vi "ADI_IMU_ADIS16448_Loop.vi"(8 "error in":errorcluster, 11 "ADI IMU DevRef":T1={"DevStatus"={"status"=FALSE, "code"=0, "source"=""}, "Handle"=0, "SPI Bus"=enum."SPI On-Board, CS0", "Device Found"=FALSE, "Device Ready"=FALSE, "Yaw Axis"=enum."Z", "AHRS Algorithm"=enum."Complementary", "Serial"=0, "Lot ID 2"=0, "Lot ID 1"=0, "Bytes Per Sample"=0, "Calibrate On Open?"=FALSE}) -> (1 "Device Found":bool)   [LabVIEW 2017, in "ADIS16448_IMU.lvlib"]
doc: "Periodically reads the ADI MXP IMU valuse and makes data available for use elsewhere in your robot project. Place this block within PeriodicTasks.vi outside any loops."
uses:
  ADIS16448_IMU.lvlib
  ADI_IMU_ADIS16448_IMUDevRef.ctl
  <vilib>/Rock Robotics/SystemInterfaces/spilib/spi_bus.ctl
panel:
  in  "Main Name":string
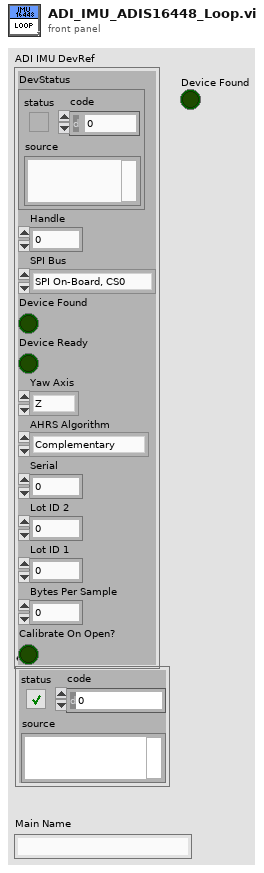
[diagram p1: front panel]
types:
  T1 = typedef "ADIS16448_IMU.lvlib/ADI_IMU_ADIS16448_IMUDevRef.ctl" = cluster{"DevStatus":errorcluster, "Handle":i32, "SPI Bus":T2, "Device Found":bool, "Device Ready":bool, "Yaw Axis":enum16{"X", "Y", "Z"}, "AHRS Algorithm":enum16{"Complementary", "Madgwick"}, "Serial":u16, "Lot ID 2":u16, "Lot ID 1":u16, "Bytes Per Sample":u16, "Calibrate On Open?":bool}
  T2 = typedef "spi_bus.ctl" = enum16{"SPI On-Board, CS0", "SPI On-Board, CS1", "SPI On-Board, CS2", "SPI On-Board, CS3", "SPI MXP", "Invalid"}
  T3 = cluster{"X Angle":dbl, "Y Angle":dbl, "Z Angle":dbl}
  T4 = enum32{"Bad", "Idle", "Run top level", "Running"}
  T5 = cluster{"X Gyro":dbl, "Y Gyro":dbl, "Z Gyro":dbl, "X Accel":dbl, "Y Accel":dbl, "Z Accel":dbl, "X Mag":dbl, "Y Mag":dbl, "Z Mag":dbl, "Pressure":dbl, "Temp":dbl}
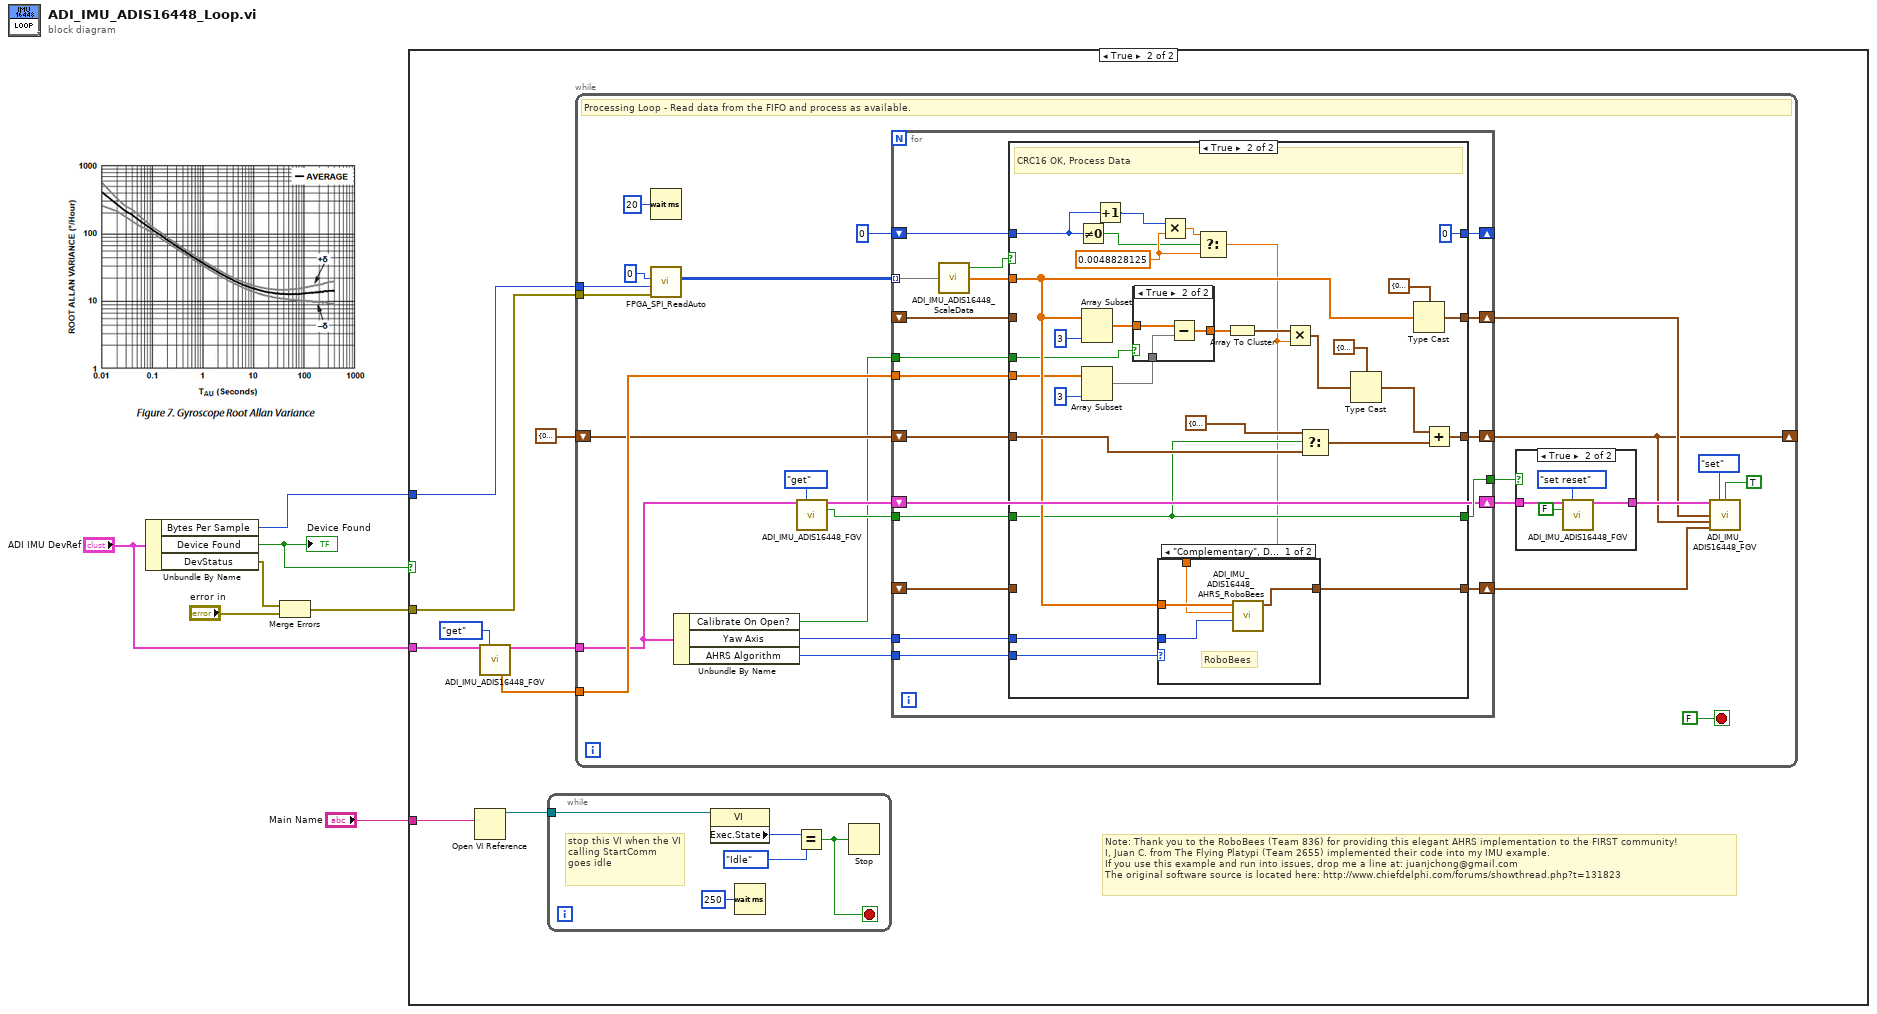
[diagram p0: block diagram]
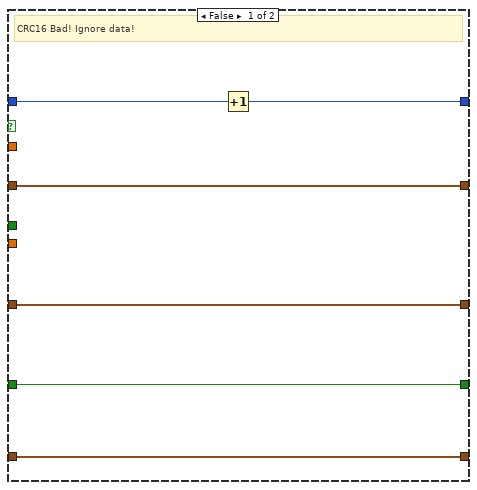
[diagram p3: hidden frame]
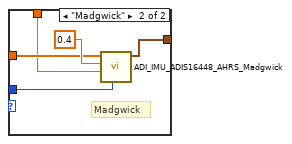
[diagram p5: hidden frame]
diagram:
  n1 = Unbundle By Name("ADI IMU DevRef") -> ("Bytes Per Sample"=w2:u16, "Device Found"=w4:bool, "DevStatus"=w5:errorcluster)
  "Device Found" <- w4
  n2 = Merge Errors(w5, "error in") -> (w1:errorcluster)
  n3 = case shown="True" w4 {
    tunnel: "Main Name" -> [_ w15]
    tunnel: "ADI IMU DevRef" -> [_ w14]
    tunnel: w2 -> [_ w10]
    tunnel: w1 -> [_ w9]
    frame False {
    }
    frame True {
      # "Note: Thank you to the RoboBees (Team 836) for providing this elegant AHRS implementation to the FIRST community!\nI, Juan C. from The Flying Platypi (Team 2655) implemented their code into my IMU example.\nIf you use this example and run into issues, drop me a line at: juanjchong@gmail.com\nThe original software source is located here: http://www.chiefdelphi.com/forums/showthread.php?t=131823"
      n4 = Open VI Reference(vi path=w15) -> (vi reference=w16:refnum<vi>)  [unwired: 1 in, 5 out]
      n5 = call "ADI_IMU_ADIS16448_FGV.vi"("ADI IMU DevRef"=w14, "Operation"=enum16{"set", "get", "set reset"}."get") -> ("ADI IMU DevRef Out"=w13:T1, "Offset Compensated Data Out"=w11:dbl[])  [unwired: 7 in, 5 out]
      n6 = while {
        tunnel: w16 -> [w18]
        stop <- w17 stop-if-true
        # "stop this VI when the VI calling StartComm goes idle"
        n7 = property class="VI"(reference=w18) -> ("Exec.State"=w20:T4)  [unwired: 1 in, 2 out]
        n8 = Wait (ms)(milliseconds to wait=u32 250) -> ()  [unwired: 1 out]
        n9 = Equal?(x=w20, y=T4."Idle" ("Execution:State")) -> (x = y?=w17:bool)
        n10 = Stop(stop? (T)=w17) -> ()
      }
      n11 = while {
        tunnel: w13 -> [w27]
        tunnel: w11 -> [w33]
        tunnel: w10 -> [w35]
        tunnel: w9 -> [w34]
        shift-right: [w25] -> _
        shift-left: T3 {"X Angle"=0.0, "Y Angle"=0.0, "Z Angle"=0.0} ("IMU Angles") -> [w31]
        stop <- FALSE stop-if-true
        # "Processing Loop - Read data from the FIFO and process as available."
        n12 = Wait (ms)(milliseconds to wait=u32 20) -> ()  [unwired: 1 out]
        n13 = call <vilib>:"FPGA_SPI_ReadAuto.vi"("error in (no error)"=w34, "Bytes per Sample"=w35, "Samples to Read"=u32 0) -> ("Data"=w30:u8[][])  [unwired: 7 in, 1 out]
        n14 = Unbundle By Name(w27) -> ("Calibrate On Open?"=w23:bool, "Yaw Axis"=w44:enum16{"X", "Y", "Z"}, "AHRS Algorithm"=w43:enum16{"Complementary", "Madgwick"})
        n15 = call "ADI_IMU_ADIS16448_FGV.vi"("ADI IMU DevRef"=w27, "Operation"=enum16{"set", "get", "set reset"}."get") -> ("ADI IMU DevRef Out"=w28:T1, "Reset Out"=w26:bool)  [unwired: 7 in, 5 out]
        n16 = for {
          tunnel: w44 -> [w61]
          tunnel: w43 -> [w60]
          tunnel: [w51] -> w38
          tunnel: w33 -> [w56]
          shift-right: [w62] -> w25
          shift-left: w31 -> [w63]
          shift-right: [w50] -> w40
          shift-left: w28 -> [w50]
          tunnel: w30 -> [w55] mode=indexing
          tunnel: w26 -> [w52]
          shift-right: [w59] -> w37
          shift-left: _ -> [w53]
          shift-right: [w48] -> _
          shift-left: 0 -> [w49]
          tunnel: w23 -> [w47]
          shift-right: [w57] -> w32
          shift-left: _ -> [w46]
          n17 = call "ADI_IMU_ADIS16448_ScaleData.vi"("Received Data"=w55) -> ("Data Array"=w58:dbl[], "Data Good?"=w54:bool)  [unwired: 3 in]
          n18 = case shown="True" w54 {
            tunnel: w63 -> [w69 w98]
            tunnel: [w69 w97] -> w62
            tunnel: w61 -> [_ w96]
            tunnel: w60 -> [_ w95]
            tunnel: [w68 w84] -> w59
            tunnel: w58 -> [_ w83]
            tunnel: [w64 w81] -> w57
            tunnel: w56 -> [_ w79]
            tunnel: w53 -> [w68 _]
            tunnel: [w67 w78] -> w51
            tunnel: w52 -> [w67 w78]
            tunnel: w49 -> [w66 w71]
            tunnel: [w65 0] -> w48
            tunnel: w47 -> [_ w70]
            tunnel: w46 -> [w64 _]
            frame False {
              # "CRC16 Bad! Ignore data!"
              n19 = Increment(x=w66) -> (x+1=w65:i32)
            }
            frame True {
              w75 = 0.0048828125
              # "CRC16 OK, Process Data"
              n20 = Not Equal To 0?(x=w71) -> (x != 0?=w74:bool)
              n21 = Array Subset(array=w83, length=3) -> (w93:dbl[])  [unwired: 1 in]
              n22 = Array Subset(array=w79, length=3) -> (w80:dbl[])  [unwired: 1 in]
              n23 = Increment(x=w71) -> (x+1=w72:i32)
              n24 = case shown="True" w70 {
                tunnel: w93 -> [w99 w102]
                tunnel: [w99 w101] -> w92
                tunnel: w80 -> [_ w100]
                frame False {
                }
                frame True {
                  n25 = Subtract(x=w102, y=w100) -> (x-y=w101:dbl[])
                }
              }
              n26 = Multiply(x=w72, y=w75) -> (x*y=w76:dbl)
              n27 = Select(t=w76, s=w74, f=w75) -> (s? t:f=w77:dbl)
              n28 = case shown="\"Complementary\", Default" w95 {
                tunnel: w83 -> [w106 w110]
                tunnel: w96 -> [w105 w109]
                tunnel: [w104 w108] -> w84
                tunnel: w77 -> [w103 w107]
                frame "Complementary", Default {
                  # "RoboBees"
                  n29 = call "ADI_IMU_ADIS16448_AHRS_RoboBees.vi"("Yaw Axis"=w105, "Delta t"=w103, "IMU Rates"=w106) -> ("Output"=w104:cluster{"Pitch":dbl, "Roll":dbl, "Yaw":dbl})  [unwired: 4 in, 3 out]
                }
                frame "Madgwick" {
                  # "Madgwick"
                  n30 = call "ADI_IMU_ADIS16448_AHRS_Madgwick.vi"("Yaw Axis"=w109, "delta t"=w107, "Beta"=0.4, "Data"=w110) -> ("Output"=w108:cluster{"Pitch":dbl, "Roll":dbl, "Yaw":dbl})  [unwired: 7 in]
                }
              }
              n31 = Array To Cluster(array=w92) -> (cluster=w91:cluster{"[0]":dbl, "[1]":dbl, "[2]":dbl})
              n32 = Multiply(x=w91, y=w77) -> (x*y=w87:cluster{"[0]":dbl, "[1]":dbl, "[2]":dbl})
              n33 = Select(t=T3 {"X Angle"=0.0, "Y Angle"=0.0, "Z Angle"=0.0} ("IMU Angles"), s=w78, f=w98) -> (s? t:f=w90:T3)
              n34 = Type Cast(type=T3 {"X Angle"=0.0, "Y Angle"=0.0, "Z Angle"=0.0} ("IMU Angles"), x=w87) -> (*(type *) &x=w88:T3)
              n35 = Type Cast(type=T5 {"X Gyro"=0.0, "Y Gyro"=0.0, "Z Gyro"=0.0, "X Accel"=0.0, "Y Accel"=0.0, "Z Accel"=0.0, "X Mag"=0.0, "Y Mag"=0.0, "Z Mag"=0.0, "Pressure"=0.0, "Temp"=0.0} ("IMU Data"), x=w83) -> (*(type *) &x=w81:T5)
              n36 = Add(x=w88, y=w90) -> (x+y=w97:T3)
            }
          }
        }
        n37 = case shown="True" w38 {
          tunnel: [w112 w115] -> w41
          tunnel: w40 -> [w112 w114]
          frame False {
          }
          frame True {
            n38 = call "ADI_IMU_ADIS16448_FGV.vi"("ADI IMU DevRef"=w114, "Operation"=enum16{"set", "get", "set reset"}."set reset", "Reset"=FALSE) -> ("ADI IMU DevRef Out"=w115:T1)  [unwired: 6 in, 6 out]
          }
        }
        n39 = call "ADI_IMU_ADIS16448_FGV.vi"("ADI IMU DevRef"=w41, "Operation"=enum16{"set", "get", "set reset"}."set", "Sensor Ready?"=TRUE, "IMU Data"=w32, "IMU Angles"=w25, "IMU AHRS"=w37) -> ()  [unwired: 3 in, 7 out]
      }
    }
  }
